vi "GetMCLBItems.vi"(0 "Ctl Refnum In":refnum<vi>, 11 "Error In":errorcluster) -> (4 "Ctl Refnum Out":refnum<vi>, 6 "MCLB Items":string[][](array[string]), 15 "Error Out":errorcluster)   [LabVIEW 2019, in "Drona.lvlib"]
doc: "This VI gets all MCLB items"
uses:
  Drona.lvlib
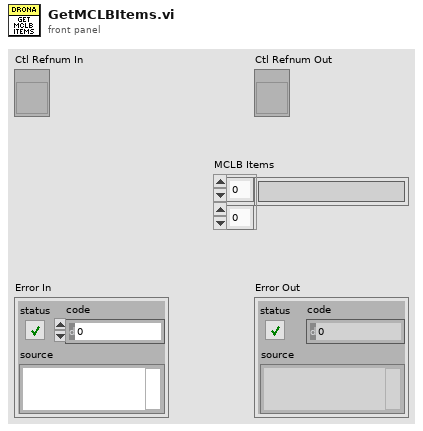
[diagram p1: front panel]
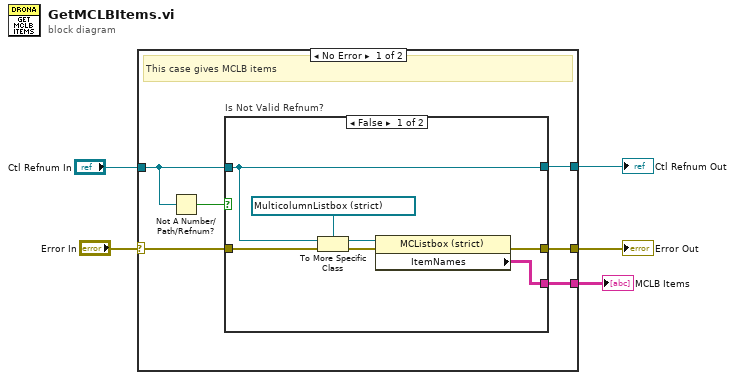
[diagram p0: block diagram]
diagram:
  n1 = case shown="No Error" "Error In" {
    selector: "Error In" -> [w11 w21]
    tunnel: "Ctl Refnum In" -> [w8 w22]
    tunnel: [w7 w22] -> w3
    tunnel: [w9 w21] -> w2
    tunnel: [w6 _] -> w1
    frame No Error {
      # "This case gives MCLB items"
      n2 = Not A Number/Path/Refnum?(number/path/refnum=w8) -> (NaN/Path/Refnum?=w10:bool)
      n3 = case "Is Not Valid Refnum?" shown="False" w10 {
        tunnel: w11 -> [w18 w20]
        tunnel: [w15 w20] -> w9
        tunnel: w8 -> [w16 w19]
        tunnel: [w16 w19] -> w7
        tunnel: [w13 _] -> w6
        frame False {
          n4 = To More Specific Class(target class=refnum<vi> refnum ("Multicolumn Listbox"), reference=w16, error in=w18) -> (specific class reference=w14:refnum<vi>, error out=w17:errorcluster)
          n5 = property class="MCListbox (strict)"(reference=w14, error in=w17) -> (error out=w15:errorcluster, "ItemNames"=w13:string[][])  [unwired: 1 out]
        }
        frame True {
        }
      }
    }
    frame Error {
      # "If error, this case pass that error messge only"
    }
  }
  "Ctl Refnum Out" <- w3
  "Error Out" <- w2
  "MCLB Items" <- w1
